vi "3D check Ant Pol Change.vi"(8 "error in (no error)":errorcluster caption="에러 입력(에러 없음)", 9 "Current Position (degree)":dbl, 10 "Target Position (deg)":dbl, 11 "Instrument Manager 입력":refnum<class "Instrument Manager.lvclass">) -> (0 "error out":errorcluster caption="에러 출력", 2 "불리언":bool, 3 "Instrument Manager 출력":refnum<class "Instrument Manager.lvclass">)   [LabVIEW 2023, in "Instrument Manager.lvclass"]
uses:
  Instrument Manager.lvclass
  Instrument Manager.lvclass/Instrument Manager.ctl
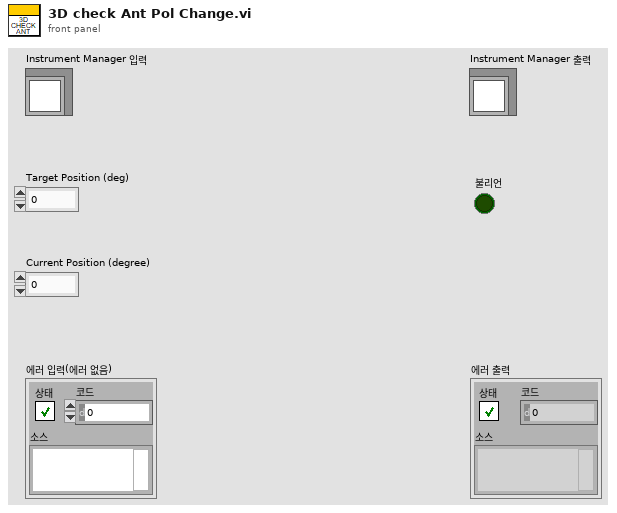
[diagram p1: front panel]
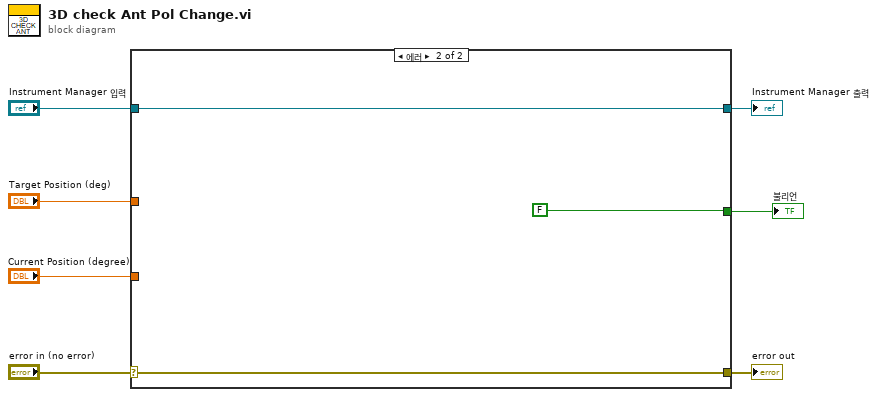
[diagram p0: block diagram]
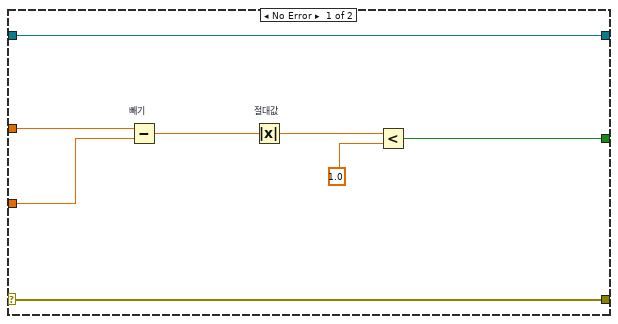
[diagram p2: hidden frame]
diagram:
  n1 = case shown="에러" "error in (no error)" {
    selector: "error in (no error)" -> [w14 w18]
    tunnel: [w14 w18] -> w6
    tunnel: [w15 w17] -> w4
    tunnel: "Instrument Manager 입력" -> [w15 w17]
    tunnel: "Target Position (deg)" -> [w13 _]
    tunnel: "Current Position (degree)" -> [w12 _]
    tunnel: [w8 FALSE] -> w1
    frame No Error {
      n2 = Subtract "빼기"(x=w13, y=w12) -> (x-y=w11:dbl)
      n3 = Absolute Value "절대값"(x=w11) -> (abs(x)=w10:dbl)
      n4 = Less?(x=w10, y=1.0) -> (x < y?=w8:bool)
    }
    frame Error {
    }
  }
  "error out" <- w6
  "Instrument Manager 출력" <- w4
  "불리언" <- w1
